vi "Control - Intake Air Measured.vi"(0 "MEP Desired [bar] (MAF w/ EGR Only)":sgl, 5 "Fuel [mg/cyc] (Fdbk)":sgl, 7 "Fuel Trim Integral Effort [mg/cyc] (VE Learn) (Fdbk) (optional)":sgl, 9 "Pre-Calculated EGR Mass Flow [kg/hr] (MAP Only)":sgl, 11 "Control Inputs":T1={"Engine Speed [RPM]"=0.0, "Engine Status"=enum."STALLED", "Load Control \nMode"=enum."Max Speed Governor", "dt(s)"=0.0, "Number of Cylinders"=0, "Engine Displacement [cc]"=0.0, "StoichAFR"=0.0, "Q.LHV Fuel [kJ/kg]"=0.0, "BattV PSU [V]"=0.0, "12V PSU [V]"=0.0, "5V PSU [V]"=0.0, "Pedal Position [%]"=0.0, "Oil Pressure [kPa]"=0.0, "Oil Temp [C]"=0.0, "Oil Level [%]"=0.0, "Engine Coolant Temp (ECT) [C]"=0.0, "Engine Coolant Pressure [kPa]"=0.0, "Rail Pressure [bar]"=0.0, "Fuel Pressure [kPa]"=0.0, "Fuel Temp [C]"=0.0, "Vacuum Pressure [kPa]"=0.0, "Throttle Position [%]"=0.0, "Cam1 Advance [CAD]"=0.0, "Cam2 Advance [CAD]"=0.0, "Cam3 Advance [CAD]"=0.0, "Cam4 Advance [CAD]"=0.0, "CA50 Control Output [CAD]"=[], "CA50 Control Output Valid"=[], "Intake Air Temp (IAT) [C]"=0.0, "Barometric Air Pressure [kPa]"=0.0, "Intake Air Rel. Humidity [%]"=0.0, "Mass Air Flow (MAF) [kg/hr]"=0.0, "Turbo Inlet Air Pressure [kPa]"=0.0, "Turbo Inlet Air Temp [C]"=0.0, "Turbo Outlet Air Pressure [kPa]"=0.0, "Turbo Outlet Air Temp [C]"=0.0, "CAC Outlet Pressure [kPa]"=0.0, "CAC Outlet Temp [C]"=0.0, "Intake Manifold Pressure (MAP) [kPa]"=0.0, "Intake Manifold Temp (MAT) [C]"=0.0, "Exhaust Manifold Pressure [kPa]"=0.0, "Exhaust Manifold Temp [C]"=0.0, "HighP EGR Cooler Outlet Pressure [kPa]"=0.0, "HighP EGR Cooler Outlet Temp [C]"=0.0, "HighP EGR Differential Pressure [kPa]"=0.0, "HighP EGR Valve Position [%]"=0.0, "Turbo Outlet Exhaust Pressure [kPa]"=0.0, "Turbo Outlet Exhaust Temp [C]"=0.0, "VGT Position 1 [%]"=0.0, "VGT Position 2 [%]"=0.0, "Turbo Speed 1 [RPM]"=0.0, "Turbo Speed 2 [RPM]"=0.0, "LowP EGR Differential Pressure [kPa]"=0.0, "LowP EGR Valve Position [%]"=0.0, "UEGO1Lambda"=0.0, "UEGO1_Hot"=FALSE, "UEGO2Lambda"=0.0, "UEGO2_Hot"=FALSE, "Knock Intensity"=[], "Knock"=[]} {"Knock Intensity" format="%.2f"; "CA50 Control Output [CAD]" format="%.2f"; "Exhaust Manifold Temp [C]" format="%#_6f"; "UEGO2Lambda" format="%.2f"; "Intake Manifold Temp (MAT) [C]" format="%#_6f"; "UEGO1Lambda" format="%.2f"}) -> (4 "Volumetric Efficiency [%]":sgl, 6 "Available Air Mass [mg/cyc]":sgl, 8 "Fresh Air Mass [mg/cyc]":sgl, 10 "Intake Charge Mass [mg/cyc]":sgl, 15 "EGR Mass [mg/cyc]":sgl)   [LabVIEW 2015, in "ECS-RT.lvlib"]
uses:
  ECS-RT.lvlib
  Typedefs/Control Inputs/Control Inputs.ctl
  Typedefs/EPT/Engine Status.ctl
  Typedefs/MISC/Load Control Mode.ctl
  Typedefs/MISC/Intake Charge Mode.ctl
  ECS-Shared.lvlib
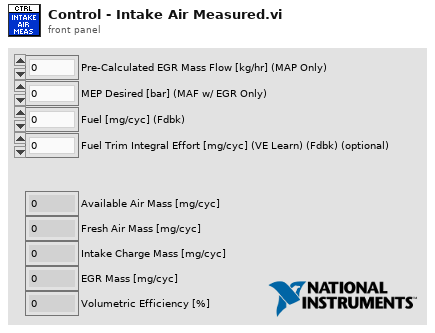
[diagram p1: front panel]
types:
  T1 = typedef "ECS-Shared.lvlib/Control Inputs.ctl" = cluster{"Engine Speed [RPM]":sgl, "Engine Status":T2, "Load Control \nMode":T3, "dt(s)":sgl, "Number of Cylinders":u8, "Engine Displacement [cc]":sgl, "StoichAFR":sgl, "Q.LHV Fuel [kJ/kg]":sgl, "BattV PSU [V]":sgl, "12V PSU [V]":sgl, "5V PSU [V]":sgl, "Pedal Position [%]":sgl, "Oil Pressure [kPa]":sgl, "Oil Temp [C]":sgl, "Oil Level [%]":sgl, "Engine Coolant Temp (ECT) [C]":sgl, "Engine Coolant Pressure [kPa]":sgl, "Rail Pressure [bar]":sgl, "Fuel Pressure [kPa]":sgl, "Fuel Temp [C]":sgl, "Vacuum Pressure [kPa]":sgl, "Throttle Position [%]":sgl, "Cam1 Advance [CAD]":sgl, "Cam2 Advance [CAD]":sgl, "Cam3 Advance [CAD]":sgl, "Cam4 Advance [CAD]":sgl, "CA50 Control Output [CAD]":sgl[], "CA50 Control Output Valid":bool[], "Intake Air Temp (IAT) [C]":sgl, "Barometric Air Pressure [kPa]":sgl, "Intake Air Rel. Humidity [%]":sgl, "Mass Air Flow (MAF) [kg/hr]":sgl, "Turbo Inlet Air Pressure [kPa]":sgl, "Turbo Inlet Air Temp [C]":sgl, "Turbo Outlet Air Pressure [kPa]":sgl, "Turbo Outlet Air Temp [C]":sgl, "CAC Outlet Pressure [kPa]":sgl, "CAC Outlet Temp [C]":sgl, "Intake Manifold Pressure (MAP) [kPa]":sgl, "Intake Manifold Temp (MAT) [C]":sgl, "Exhaust Manifold Pressure [kPa]":sgl, "Exhaust Manifold Temp [C]":sgl, "HighP EGR Cooler Outlet Pressure [kPa]":sgl, "HighP EGR Cooler Outlet Temp [C]":sgl, "HighP EGR Differential Pressure [kPa]":sgl, "HighP EGR Valve Position [%]":sgl, "Turbo Outlet Exhaust Pressure [kPa]":sgl, "Turbo Outlet Exhaust Temp [C]":sgl, "VGT Position 1 [%]":sgl, "VGT Position 2 [%]":sgl, "Turbo Speed 1 [RPM]":sgl, "Turbo Speed 2 [RPM]":sgl, "LowP EGR Differential Pressure [kPa]":sgl, "LowP EGR Valve Position [%]":sgl, "UEGO1Lambda":sgl, "UEGO1_Hot":bool, "UEGO2Lambda":sgl, "UEGO2_Hot":bool, "Knock Intensity":sgl[], "Knock":bool[]}
  T2 = typedef "ECS-Shared.lvlib/Engine Status.ctl" = enum16{"OFF", "STALLED", "CRANKING", "RUNNING", "ACCEL", "DECEL", "SAFE"}
  T3 = typedef "ECS-Shared.lvlib/Load Control Mode.ctl" = enum16{"No Governor", "Min Speed Governor", "Max Speed Governor"}
  T4 = typedef "ECS-Shared.lvlib/Intake Charge Mode.ctl" = enum32{"MAF Only (No EGR)", "MAF Only (EGR)", "MAP Only (No EGR)", "MAP Only (EGR)", "MAF + MAP (EGR)"}
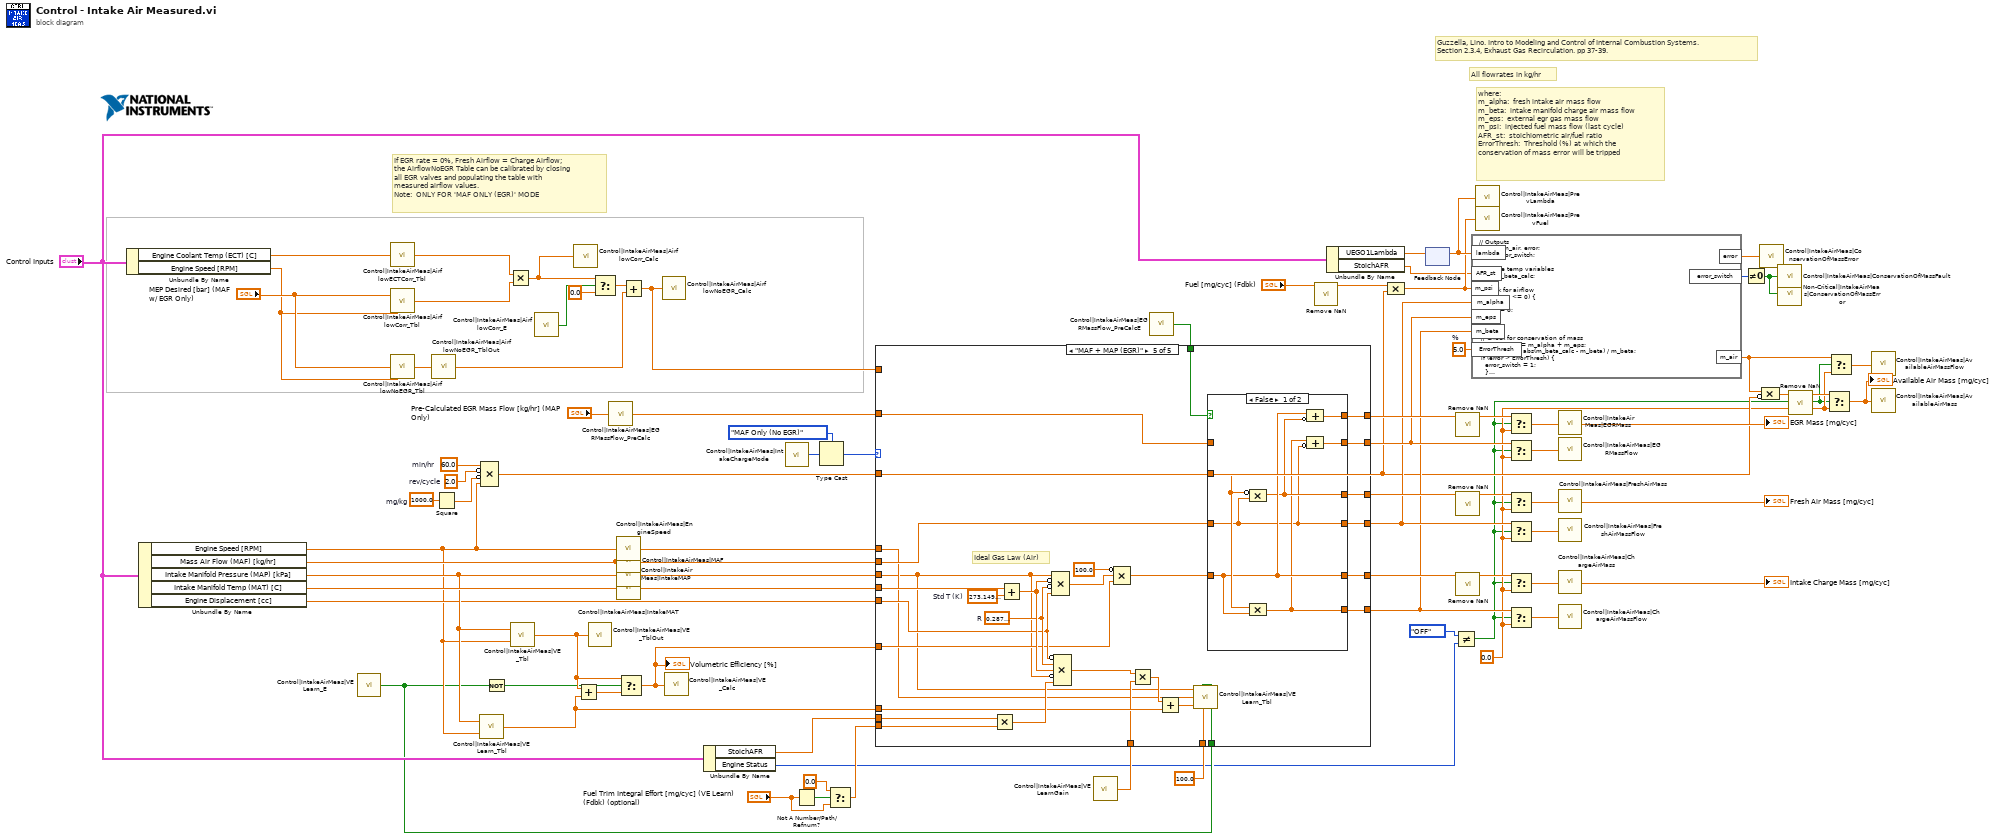
[diagram p0: block diagram]
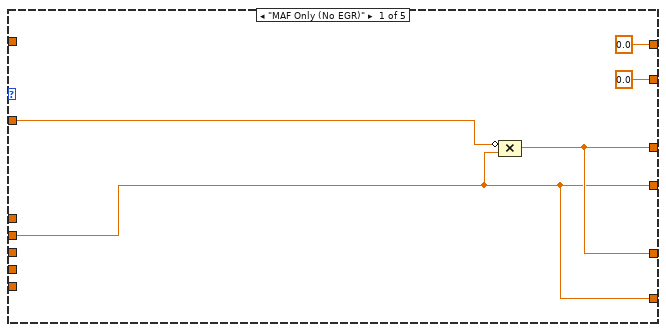
[diagram p2: hidden frame]
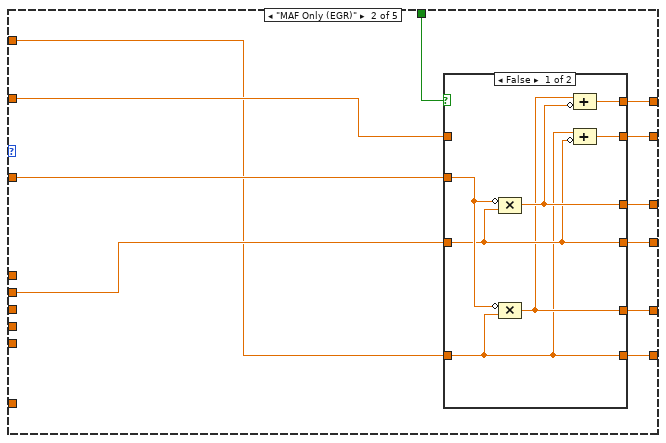
[diagram p3: hidden frame]
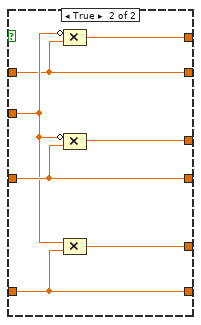
[diagram p4: hidden frame]
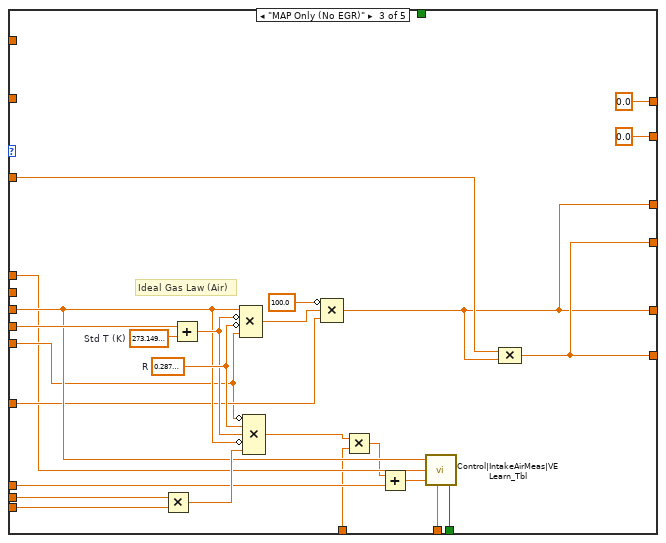
[diagram p5: hidden frame]
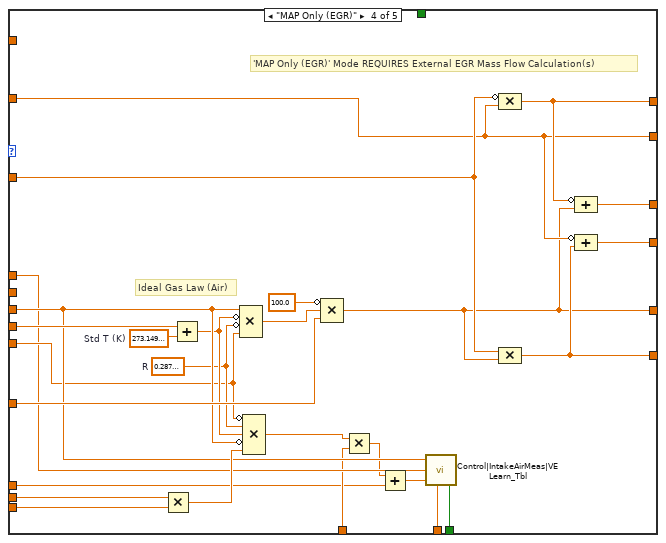
[diagram p6: hidden frame]
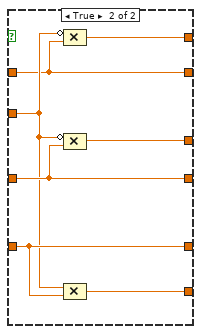
[diagram p7: hidden frame]
diagram:
  w2 = sgl 0.0 ("f")
  w54 = 5.0  # %
  w59 = sgl 60.0  # min/hr
  w60 = sgl 2.0  # rev/cycle
  w58 = sgl 1000.0  # mg/kg
  # "where:\nm_alpha:  fresh intake air mass flow\nm_beta:  intake manifold charge air mass flow\nm_eps:  external egr gas mass flow\nm_psi:  injected fuel mass flow (last cycle)\nAFR_st:  stoichiometric air/fuel ratio\nErrorThresh:  Threshold (%) at which the\nconservation of mass error will be tripped"
  # "All flowrates in kg/hr"
  # "Guzzella, Lino. Intro to Modeling and Control of Internal Combustion Systems.  \nSection 2.3.4, Exhaust Gas Recirculation. pp 37-39."
  # "If EGR rate = 0%, Fresh Airflow = Charge Airflow;\nthe AirflowNoEGR Table can be calibrated by closing\nall EGR valves and populating the table with\nmeasured airflow values.\nNote:  ONLY FOR 'MAF ONLY (EGR)' MODE"
  n1 = Unbundle By Name("Control Inputs") -> ("Engine Coolant Temp (ECT) [C]"=w64:sgl, "Engine Speed [RPM]"=w57:sgl)
  n2 = Unbundle By Name("Control Inputs") -> ("Engine Speed [RPM]"=w42:sgl, "Mass Air Flow (MAF) [kg/hr]"=w50:sgl, "Intake Manifold Pressure (MAP) [kPa]"=w44:sgl, "Intake Manifold Temp (MAT) [C]"=w49:sgl, "Engine Displacement [cc]"=w43:sgl)
  n3 = call "Control|IntakeAirMeas|VELearn_E"() -> ("Value"=w24:bool)
  n4 = call "Control|IntakeAirMeas|AirflowECTCorr_Tbl"("X Index"=w64) -> ("Y"=w69:sgl)
  n5 = call "Control|IntakeAirMeas|AirflowCorr_Tbl"("Y Index"=w57, "X Index"="MEP Desired [bar] (MAF w/ EGR Only)") -> ("Z"=w68:sgl)
  n6 = call "Control|IntakeAirMeas|AirflowNoEGR_Tbl"("Y Index"=w57, "X Index"="MEP Desired [bar] (MAF w/ EGR Only)") -> ("Z"=w71:sgl)
  n7 = call "Control|IntakeAirMeas|AirflowNoEGR_TblOut"("Value"=w71) -> ()
  n8 = Square(x=w58) -> (x^2=w61:sgl)
  n9 = call "Control|IntakeAirMeas|VELearn_Tbl"("Y Index"=w42, "X Index"=w44) -> ("Z"=w25:sgl)
  n10 = Compound Arithmetic op=MULTIPLY(w59, invert w60, invert w61, w42) -> (w7:sgl)
  n11 = Not(x=w24) -> (.not. x?=w23:bool)
  n12 = Multiply(x=w69, y=w68) -> (x*y=w70:sgl)
  n13 = call "Control|IntakeAirMeas|VE_Tbl"("Y Index"=w42, "X Index"=w44) -> ("Z"=w27:sgl)
  n14 = call "Control|IntakeAirMeas|AirflowCorr_E"() -> ("Value"=w66:bool)
  n15 = call "Control|IntakeAirMeas|AirflowCorr_Calc"("Value"=w70) -> ()
  n16 = Add(x=w27, y=w25) -> (x+y=w28:sgl)
  n17 = call "Control|IntakeAirMeas|VE_TblOut"("Value"=w27) -> ()
  n18 = Select(t=w70, s=w66, f=sgl 0.0) -> (s? t:f=w67:sgl)
  n19 = call "Control|IntakeAirMeas|EGRMassFlow_PreCalc"("Value"="Pre-Calculated EGR Mass Flow [kg/hr] (MAP Only)") -> ()
  n20 = call "Control|IntakeAirMeas|EngineSpeed"("Value"=w42) -> ()
  n21 = call "Control|IntakeAirMeas|MAF"("Value"=w50) -> ()
  n22 = call "Control|IntakeAirMeas|IntakeMAP"("Value"=w44) -> ()
  n23 = call "Control|IntakeAirMeas|IntakeMAT"("Value"=w49) -> ()
  n24 = Select(t=w27, s=w23, f=w28) -> (s? t:f=w38:sgl)
  "Volumetric Efficiency [%]" <- w38
  n25 = Add(x=w67, y=w71) -> (x+y=w63:sgl)
  n26 = call "Control|IntakeAirMeas|AirflowNoEGR_Calc"("Value"=w63) -> ()
  n27 = call "Control|IntakeAirMeas|VE_Calc"("Value"=w38) -> ()
  n28 = Unbundle By Name("Control Inputs") -> ("StoichAFR"=w30:sgl, "Engine Status"=w8:T2)
  n29 = call "Control|IntakeAirMeas|IntakeChargeMode"() -> ("Value"=w74:u32)
  n30 = Not A Number/Path/Refnum?(number/path/refnum="Fuel Trim Integral Effort [mg/cyc] (VE Learn) (Fdbk) (optional)") -> (NaN/Path/Refnum?=w36:bool)
  n31 = Type Cast(type=Intake_Charge_Mode."MAF Only (No EGR)" ("EGR Estimation Mode"), x=w74) -> (*(type *) &x=w72:T4)
  n32 = Select(t=sgl 0.0, s=w36, f="Fuel Trim Integral Effort [mg/cyc] (VE Learn) (Fdbk) (optional)") -> (s? t:f=w34:sgl)
  n33 = call "Control|IntakeAirMeas|VELearnGain"() -> ("Value"=w22:sgl)
  n34 = call "Control|IntakeAirMeas|EGRMassFlow_PreCalcE"() -> ("Value"=w47:bool)
  n35 = case shown="\"MAF + MAP (EGR)\"" w72 {
    tunnel: [sgl 0.0 ("EGR Mass Flow [kg/hr] (optional for MAF, MAF+MAP modes)") w86 sgl 0.0 ("EGR Mass Flow [kg/hr] (optional for MAF, MAF+MAP modes)") w147 w183] -> w16
    tunnel: [w75 w90 w123 w150 w187] -> w15
    tunnel: [w76 w88 w122 w151 w185] -> w41
    tunnel: w63 -> [_ w81 _ _ _]
    tunnel: [w75 w87 w123 w148 w184] -> w11
    tunnel: [w76 w89 w122 w146 w186] -> w39
    tunnel: [sgl 0.0 w85 sgl 0.0 w149 w182] -> w40
    tunnel: "Pre-Calculated EGR Mass Flow [kg/hr] (MAP Only)" -> [_ w84 _ w147 w181]
    tunnel: w7 -> [w79 w82 w126 w152 w180]
    tunnel: w50 -> [w75 w83 _ _ w159]
    tunnel: w44 -> [_ _ w114 w140 w157]
    tunnel: w49 -> [_ _ w121 w153 w171]
    tunnel: w43 -> [_ _ w112 w137 w172]
    tunnel: w38 -> [_ _ w113 w141 w170]
    tunnel: w47 -> [_ w80 _ _ w179]
    tunnel: w42 -> [_ _ w111 w136 w158]
    tunnel: w24 -> [_ _ w119 w143 w162]
    tunnel: sgl 100.0 ("Value") -> [_ _ w120 w142 w163]
    tunnel: w34 -> [_ _ w118 w144 w169]
    tunnel: w30 -> [_ _ w110 w135 w167]
    tunnel: w22 -> [_ _ w106 w133 w161]
    tunnel: w25 -> [_ _ w108 w130 w164]
    frame "MAF Only (No EGR)" {
      n36 = Compound Arithmetic op=MULTIPLY(invert w79, w75) -> (w76:sgl)
    }
    frame "MAF Only (EGR)" {
      n37 = case shown="False" w80 {
        tunnel: w83 -> [w93 w103]
        tunnel: w84 -> [_ w100]
        tunnel: [w93 w103] -> w90
        tunnel: [w92 w99] -> w89
        tunnel: w82 -> [w97 w101]
        tunnel: [w94 w104] -> w88
        tunnel: [w91 w98] -> w87
        tunnel: [w96 w100] -> w86
        tunnel: [w95 w102] -> w85
        tunnel: w81 -> [w91 w98]
        frame False {
          n38 = Compound Arithmetic op=MULTIPLY(invert w97, w93) -> (w94:sgl)
          n39 = Compound Arithmetic op=MULTIPLY(invert w97, w91) -> (w92:sgl)
          n40 = Compound Arithmetic op=ADD(w92, invert w94) -> (w95:sgl)
          n41 = Compound Arithmetic op=ADD(w91, invert w93) -> (w96:sgl)
        }
        frame True {
          n42 = Compound Arithmetic op=MULTIPLY(invert w101, w100) -> (w102:sgl)
          n43 = Compound Arithmetic op=MULTIPLY(invert w101, w103) -> (w104:sgl)
          n44 = Compound Arithmetic op=MULTIPLY(w101, w98) -> (w99:sgl)
        }
      }
    }
    frame "MAP Only (No EGR)" {
      w117 = sgl 0.287  # R
      w129 = sgl 273.15  # Std T (K)
      # "Ideal Gas Law (Air)"
      n45 = Multiply(x=w110, y=w118) -> (x*y=w115:sgl)
      n46 = Add(x=w121, y=w129) -> (x+y=w116:sgl)
      n47 = Compound Arithmetic op=MULTIPLY(w114, invert w116, invert w117, w112) -> (w127:sgl)
      n48 = Compound Arithmetic op=MULTIPLY(invert w112, w117, w116, invert w114, w115) -> (w107:sgl)
      n49 = Compound Arithmetic op=MULTIPLY(invert sgl 100.0 ("y"), w127, w113) -> (w122:sgl)
      n50 = Multiply(x=w107, y=w106) -> (x*y=w105:sgl)
      n51 = Add(x=w105, y=w108) -> (x+y=w109:sgl)
      n52 = call "Control|IntakeAirMeas|VELearn_Tbl"("X"=w114, "Adapt"=w119, "Y"=w111, "Z"=w109, "%/100"=w120) -> ()  [unwired: 1 in]
      n53 = Compound Arithmetic op=MULTIPLY(w126, w122) -> (w123:sgl)
    }
    frame "MAP Only (EGR)" {
      w138 = sgl 0.287  # R
      w156 = sgl 273.15  # Std T (K)
      # "'MAP Only (EGR)' Mode REQUIRES External EGR Mass Flow Calculation(s)"
      # "Ideal Gas Law (Air)"
      n54 = Multiply(x=w135, y=w144) -> (x*y=w145:sgl)
      n55 = Add(x=w153, y=w156) -> (x+y=w139:sgl)
      n56 = Compound Arithmetic op=MULTIPLY(w140, invert w139, invert w138, w137) -> (w154:sgl)
      n57 = Compound Arithmetic op=MULTIPLY(invert w137, w138, w139, invert w140, w145) -> (w132:sgl)
      n58 = Compound Arithmetic op=MULTIPLY(invert sgl 100.0 ("y"), w154, w141) -> (w146:sgl)
      n59 = Multiply(x=w132, y=w133) -> (x*y=w131:sgl)
      n60 = Add(x=w131, y=w130) -> (x+y=w134:sgl)
      n61 = call "Control|IntakeAirMeas|VELearn_Tbl"("X"=w140, "Adapt"=w143, "Y"=w136, "Z"=w134, "%/100"=w142) -> ()  [unwired: 1 in]
      n62 = Compound Arithmetic op=MULTIPLY(invert w152, w147) -> (w149:sgl)
      n63 = Compound Arithmetic op=MULTIPLY(w152, w146) -> (w148:sgl)
      n64 = Compound Arithmetic op=ADD(invert w149, w146) -> (w151:sgl)
      n65 = Compound Arithmetic op=ADD(invert w147, w148) -> (w150:sgl)
    }
    frame "MAF + MAP (EGR)" {
      w173 = sgl 0.287  # R
      w178 = sgl 273.15  # Std T (K)
      # "Ideal Gas Law (Air)"
      # "Ideal Gas Law (Air)"
      n66 = Multiply(x=w167, y=w169) -> (x*y=w175:sgl)
      n67 = Add(x=w171, y=w178) -> (x+y=w174:sgl)
      n68 = Compound Arithmetic op=MULTIPLY(w157, invert w174, invert w173, w172) -> (w176:sgl)
      n69 = Compound Arithmetic op=MULTIPLY(invert w172, w173, w174, invert w157, w175) -> (w160:sgl)
      n70 = Compound Arithmetic op=MULTIPLY(invert sgl 100.0 ("y"), w176, w170) -> (w168:sgl)
      n71 = Multiply(x=w160, y=w161) -> (x*y=w165:sgl)
      n72 = Add(x=w165, y=w164) -> (x+y=w166:sgl)
      n73 = call "Control|IntakeAirMeas|VELearn_Tbl"("X"=w157, "Adapt"=w162, "Y"=w158, "Z"=w166, "%/100"=w163) -> ()  [unwired: 1 in]
      n74 = case shown="False" w179 {
        tunnel: w168 -> [w191 w199]
        tunnel: w159 -> [w188 w198]
        tunnel: w181 -> [_ w195]
        tunnel: [w188 w198] -> w187
        tunnel: [w191 w199] -> w186
        tunnel: w180 -> [w194 w196]
        tunnel: [w190 w201] -> w185
        tunnel: [w189 w200] -> w184
        tunnel: [w193 w195] -> w183
        tunnel: [w192 w197] -> w182
        frame False {
          n75 = Compound Arithmetic op=MULTIPLY(invert w194, w188) -> (w190:sgl)
          n76 = Compound Arithmetic op=MULTIPLY(w194, w191) -> (w189:sgl)
          n77 = Compound Arithmetic op=ADD(w191, invert w190) -> (w192:sgl)
          n78 = Compound Arithmetic op=ADD(w189, invert w188) -> (w193:sgl)
        }
        frame True {
          n79 = Compound Arithmetic op=MULTIPLY(invert w196, w195) -> (w197:sgl)
          n80 = Compound Arithmetic op=MULTIPLY(invert w196, w198) -> (w201:sgl)
          n81 = Compound Arithmetic op=MULTIPLY(w196, w199) -> (w200:sgl)
        }
      }
    }
  }
  n82 = call "Remove NaN.vi"("Value In"="Fuel [mg/cyc] (Fdbk)") -> ("Value Out"=w32:sgl)  [unwired: 10 in]
  n83 = Unbundle By Name("Control Inputs") -> ("UEGO1Lambda"=w55:sgl, "StoichAFR"=w21:sgl)
  n84 = Compound Arithmetic op=MULTIPLY(w32, w7) -> (w45:sgl)
  n85 = feedback-in #1(w55) -> ()
  n86 = feedback #1() -> (w46:sgl)  [unwired: 1 in]
  n87 = Not Equal?(x=Engine_Status."OFF" ("Engine Status"), y=w8) -> (x != y?=w1:bool)
  n88 = call "Remove NaN.vi"("Value In"=w40) -> ("Value Out"=w31:sgl)  [unwired: 10 in]
  n89 = call "Remove NaN.vi"("Value In"=w41) -> ("Value Out"=w19:sgl)  [unwired: 10 in]
  n90 = call "Remove NaN.vi"("Value In"=w39) -> ("Value Out"=w13:sgl)  [unwired: 10 in]
  n91 = formula code="// Outputs\nfloat32 m_air, error;\nuInt8 error_switch;\n\n// Create temp variables\nfloat m_beta_calc;\n\n//Check for airflow\nif (m_beta <= 0) {\n error = 0;\n m_air = 0;\n }\nelse {\n\n // Check for conservation of mass\n m_beta_calc = m_alpha + m_eps;\n error = 100 * abs(m_beta_calc - m_beta) / m_beta;\n if (error > ErrorThresh) {\n   error_switch = 1;\n   }\n else {\n   error_switch = 0;\n   }\n\n // Calculate Available air mass flow\n if (lambda < 1) {\n   m_air = m_alpha;\n    }\n else {\n   m_air = m_alpha + ((m_eps*(lambda-1)*AFR_st*m_psi)/(m_beta+m_psi));\n   }\n }"("m_psi"=w45, "m_beta"=w11, "lambda"=w46, "AFR_st"=w21, "m_eps"=w16, "m_alpha"=w15, "ErrorThresh"=w54) -> ("m_air"=w4:sgl, "error_switch"=w52:u8, "error"=w53:sgl)
  n92 = call "Control|IntakeAirMeas|PrevLambda"("Value"=w46) -> ()
  n93 = call "Control|IntakeAirMeas|PrevFuel"("Value"=w45) -> ()
  n94 = Select(t=w31, s=w1, f=w2) -> (s? t:f=w20:sgl)
  "EGR Mass [mg/cyc]" <- w20
  n95 = Select(t=w16, s=w1, f=w2) -> (s? t:f=w17:sgl)
  n96 = Select(t=w19, s=w1, f=w2) -> (s? t:f=w18:sgl)
  "Fresh Air Mass [mg/cyc]" <- w18
  n97 = Select(t=w15, s=w1, f=w2) -> (s? t:f=w14:sgl)
  n98 = Select(t=w13, s=w1, f=w2) -> (s? t:f=w12:sgl)
  "Intake Charge Mass [mg/cyc]" <- w12
  n99 = Select(t=w11, s=w1, f=w2) -> (s? t:f=w10:sgl)
  n100 = call "Control|IntakeAirMeas|EGRMass"("Value"=w20) -> ()
  n101 = call "Control|IntakeAirMeas|EGRMassFlow"("Value"=w17) -> ()
  n102 = call "Control|IntakeAirMeas|FreshAirMass"("Value"=w18) -> ()
  n103 = call "Control|IntakeAirMeas|FreshAirMassFlow"("Value"=w14) -> ()
  n104 = call "Control|IntakeAirMeas|ChargeAirMass"("Value"=w12) -> ()
  n105 = call "Control|IntakeAirMeas|ChargeAirMassFlow"("Value"=w10) -> ()
  n106 = Not Equal To 0?(x=w52) -> (x != 0?=w51:bool)
  n107 = call "Control|IntakeAirMeas|ConservationOfMassError"("Value"=w53) -> ()
  n108 = Compound Arithmetic op=MULTIPLY(w4, invert w7) -> (w56:sgl)
  n109 = call "Control|IntakeAirMeas|ConservationOfMassFault"("Value"=w51) -> ()
  n110 = call "Non-Critical|IntakeAirMeas|ConservationOfMassError"("Fault"=w51) -> ()  [unwired: 2 in]
  n111 = call "Remove NaN.vi"("Value In"=w56) -> ("Value Out"=w6:sgl)  [unwired: 10 in]
  n112 = Select(t=w6, s=w1, f=w2) -> (s? t:f=w5:sgl)
  "Available Air Mass [mg/cyc]" <- w5
  n113 = Select(t=w4, s=w1, f=w2) -> (s? t:f=w3:sgl)
  n114 = call "Control|IntakeAirMeas|AvailableAirMassFlow"("Value"=w3) -> ()
  n115 = call "Control|IntakeAirMeas|AvailableAirMass"("Value"=w5) -> ()
